vi "Probe Frame SR Read.vi"() -> ()   [LabVIEW 2026]
doc: "Probe: can a Node inside a Case frame read a shift-register net declared at loop level (net 240.acc), without an explicit case tunnel? Frame True runs Add(SR, Step) and writes the frame-level Out tunnel; frame False passes the SR value straight through (the pattern proven in round3 v2). If this validates and converts, state machines can read data registers directly inside their frames."
panel:
  out "Iterations":i32
  out "Final Value":dbl
  in  "Max Iterations":i32=3
  in  "Mode":bool=TRUE
  in  "Step":dbl=3.0
  in  "Start":dbl=2.0
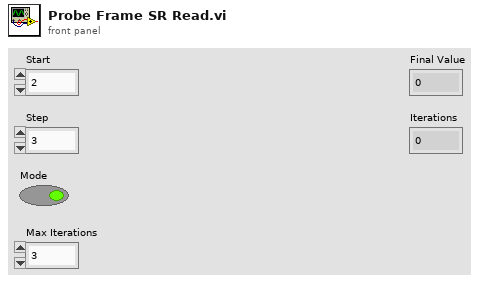
[diagram p1: front panel]
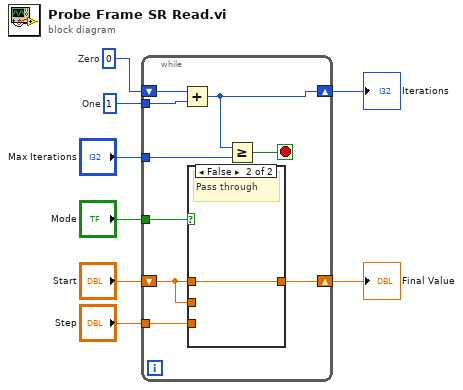
[diagram p0: block diagram]
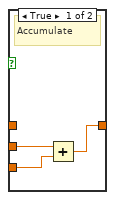
[diagram p2: hidden frame]
diagram:
  w4 = 1  # One
  w5 = 0  # Zero
  n1 = while {
    tunnel: "Step" -> [w12]
    tunnel: "Max Iterations" -> [w14]
    shift-right: [w10] -> w2
    shift-left: "Start" -> [w11]
    shift-right: [w15] -> w1
    shift-left: w5 -> [w17]
    tunnel: w4 -> [w16]
    tunnel: "Mode" -> [w9]
    stop <- w13 stop-if-true
    n2 = Add(x=w17, y=w16) -> (x+y=w15:i32)
    n3 = case shown="False" w9 {
      tunnel: w12 -> [w19 _]
      tunnel: w11 -> [w20 _]
      tunnel: [w18 w21] -> w10
      tunnel: w11 -> [_ w21]
      frame True {
        # "Accumulate"
        n4 = Add(x=w20, y=w19) -> (x+y=w18:dbl)
      }
      frame False {
        # "Pass through"
      }
    }
    n5 = Greater Or Equal?(x=w15, y=w14) -> (x >= y?=w13:bool)
  }
  "Final Value" <- w2
  "Iterations" <- w1
